vi "Verbosity Test.vi"(8 "error in (no error)":errorcluster) -> (0 "error out":errorcluster)   [LabVIEW 2020]
uses:
  classes/Assert/Assert True.vi
  classes/Assert/Assert False.vi
  classes/Assert/Assert Error.vi
  classes/Assert/Assert Not Error.vi
  classes/Assert/Assert Equal Value_Variant.vi
  classes/Assert/Assert Greater_Variant.vi
  classes/Assert/Assert Less Or Equal_Variant.vi
  classes/Test/Test.lvclass
  classes/Assert/Assert.lvclass
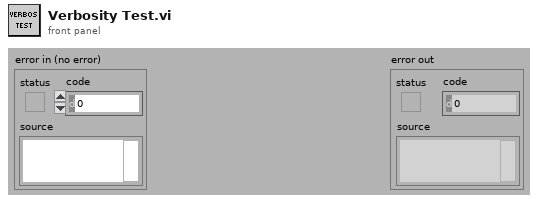
[diagram p1: front panel]
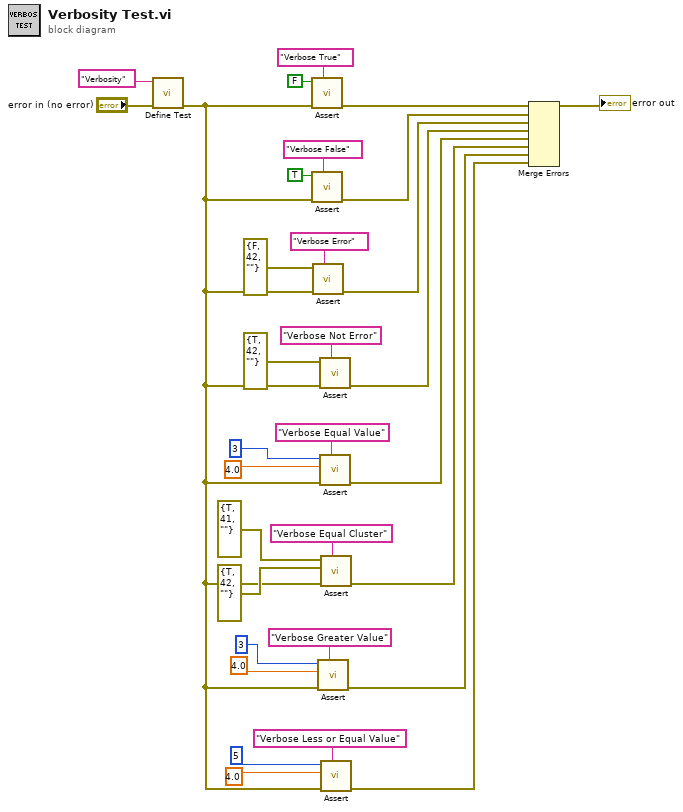
[diagram p0: block diagram]
diagram:
  n1 = call "Define Test.vi"("error in (no error)"="error in (no error)", "Label (VI Title)"="Verbosity" ("Label")) -> ("error out"=w5:errorcluster)  [unwired: 8 in, 1 out]
  n2 = call-poly "Assert.vi"("Label"="Verbose True", "error in (no error)"=w5, "True?"=FALSE) -> ("error out"=w28:errorcluster)  [unwired: 7 in, 1 out]
  n3 = call-poly "Assert.vi"("Label"="Verbose False", "error in (no error)"=w5, "False?"=TRUE) -> ("error out"=w24:errorcluster)  [unwired: 7 in, 1 out]
  n4 = call-poly "Assert.vi"("Label"="Verbose Error", "error in (no error)"=w5, "Error?"=errorcluster {"status"=FALSE, "code"=42, "source"=""}) -> ("error out"=w22:errorcluster)  [unwired: 7 in, 1 out]
  n5 = call-poly "Assert.vi"("Label"="Verbose Greater Value", "error in (no error)"=w5, "Y"=4.0, "X"=3) -> ("error out"=w13:errorcluster)  [unwired: 6 in, 1 out]
  n6 = call-poly "Assert.vi"("Label"="Verbose Not Error", "error in (no error)"=w5, "Not Error?"=errorcluster {"status"=TRUE, "code"=42, "source"=""}) -> ("error out"=w20:errorcluster)  [unwired: 7 in, 1 out]
  n7 = call-poly "Assert.vi"("Label"="Verbose Equal Value", "error in (no error)"=w5, "Y"=4.0, "X"=3) -> ("error out"=w4:errorcluster)  [unwired: 6 in, 1 out]
  n8 = call-poly "Assert.vi"("Label"="Verbose Equal Cluster", "error in (no error)"=w5, "Y"=errorcluster {"status"=TRUE, "code"=42, "source"=""} ("Not Error?"), "X"=errorcluster {"status"=TRUE, "code"=41, "source"=""} ("Not Error?")) -> ("error out"=w7:errorcluster)  [unwired: 6 in, 1 out]
  n9 = call-poly "Assert.vi"("Label"="Verbose Less or Equal Value", "error in (no error)"=w5, "Y"=4.0, "X"=5) -> ("error out"=w17:errorcluster)  [unwired: 6 in, 1 out]
  n10 = Merge Errors(w28, w24, w22, w20, w4, w7, w13, w17) -> (→"error out":errorcluster)
